vi "Flatten Buffer Configuration.vi"(11 "Buffer Configuration":T1) -> (3 "Flattened Configuration":u8[](array[numeric]) format="%.0x")   [LabVIEW 2021, in "CIF_Iceoryx_PCAP_Universal.lvclass"]
uses:
  CIF_Iceoryx_PCAP_Universal.lvclass
  Typedef/Buffer Configuration Data.ctl
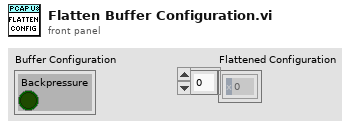
[diagram p1: front panel]
types:
  T1 = typedef "CIF_Iceoryx_PCAP_Universal.lvclass/Buffer Configuration Data.ctl" = cluster{"Backpressure":bool}
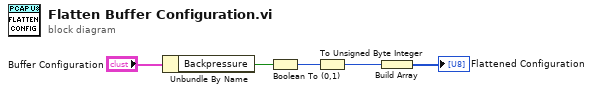
[diagram p0: block diagram]
diagram:
  n1 = Unbundle By Name("Buffer Configuration") -> ("Backpressure"=w3:bool)
  n2 = Boolean To (0,1)(Boolean=w3) -> (0, 1=w2:i16)
  n3 = To Unsigned Byte Integer(number=w2) -> (unsigned 8bit integer=w1:u8)
  n4 = Build Array(w1) -> (→"Flattened Configuration":u8[])
